vi "Create.vi"(8 "error in":errorcluster) -> (0 "error out":errorcluster, 3 "ToastBuilder out":refnum<class "ToastBuilder.lvclass">)   [LabVIEW 2026, in "ToastNotification.lvlib" / "ToastBuilder.lvclass"]
doc: "Create a new ToastBuilder owning a native ToastContentBuilder reference. Call once before composition methods and close the returned builder after use. With an incoming error, return a default uninitialized builder and preserve the error. The internal release step operates on the new default instance; this VI has no existing-builder input and is not an in-place reinitialization API."
uses:
  ToastBuilder.lvclass
  ToastBuilder.lvclass/ToastBuilder.ctl
  Read Builder Reference.vi
  Write Builder Reference.vi
  Toast Native/Toast Native.lvlib
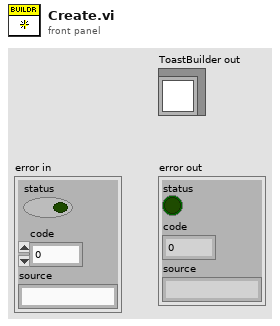
[diagram p1: front panel]
types:
  T1 = typedef "ToastNotification.lvlib/ToastBuilder.lvclass/Builder Reference.ctl" = refnum<k24>
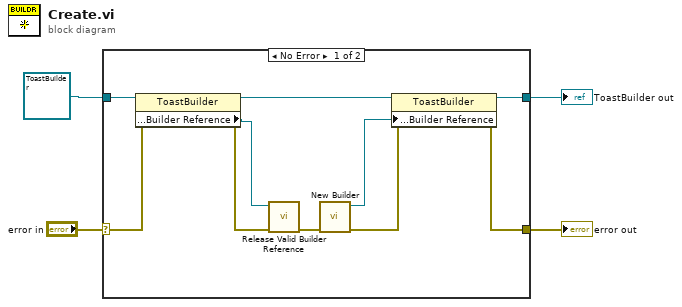
[diagram p0: block diagram]
diagram:
  n1 = case shown="No Error" "error in" {
    selector: "error in" -> [w12 w15]
    tunnel: refnum<class "ToastBuilder.lvclass"> refnum -> [w14 w16]
    tunnel: [w11 w16] -> w2
    tunnel: [w9 w15] -> w1
    frame No Error {
      n2 = property class="ToastBuilder"(reference=w14, error in=w12) -> (reference out=w13:refnum<class "ToastBuilder.lvclass">, error out=w10:errorcluster, "Public:Properties:Builder Reference"=w5:T1)
      n3 = call "Release Valid Builder Reference.vi"("error in (no error)"=w10, "reference"=w5) -> ("error out"=w8:errorcluster)  [unwired: 9 in]
      n4 = call "New Builder.vi"("error in (no error)"=w8) -> ("error out"=w7:errorcluster, "new reference"=w6:refnum<k24>)  [unwired: 9 in]
      n5 = property class="ToastBuilder"(reference=w13, error in=w7, "Public:Properties:Builder Reference"=w6) -> (reference out=w11:refnum<class "ToastBuilder.lvclass">, error out=w9:errorcluster)
    }
    frame Error {
    }
  }
  "ToastBuilder out" <- w2
  "error out" <- w1
